vi "Measurement UI.vi"() -> ()   [LabVIEW 2025, in "Automotive Vision UI.lvlib"]
uses:
  Automotive Vision UI.lvlib
  <vilib>/gRPC/LabVIEW gRPC Library/Shared/grpcId.ctl
  <vilib>/vision/Image Controls.llb/IMAQ Image.ctl
  Automotive-Vision-OOBService_client/RPC Messages/hwval_BoolRequest.ctl
  Automotive-Vision-OOBService_client/RPC Messages/hwval_ExportRequest.ctl
  Automotive-Vision-OOBService_client/RPC Messages/hwval_ExportTypeRequest.ctl
  Automotive-Vision-OOBService_client/RPC Messages/hwval_ExportFileType.ctl
  <vilib>/gRPC/LabVIEW gRPC Library/grpc-lvsupport-release.lvlib
  Automotive-Vision-OOBService_client/Automotive-Vision-OOBService_client.lvlib
panel:
  in  "HELP":bool
  out "WIDTH":u64
  out "HEIGHT":u64
  out "Numeric":i32
  out "error out":errorcluster
  in  "GRPC status":string
  out "OOB gRPC Port":i32
  in  "BITFILE":string="IMAGE RESOLUTION: 800x600 - RAW12"
  in  "SERIAL (SI) CHANNEL":u32(ring) items=["SI0", "SI1", "SI2", "SI3"]
  out "Available SI Devices":string[][](array[string])
  in  "RIO HANDLER":string
  in  "AUTO. VISION DEVICE":u32(ring) items=["PXI1Slot2", "PXI1Slot5"]
  out "BYTES ACQUIRED":u64 format="%#.2p"
  out "ERROR":bool
  out "IMAGE PIXEL DATA":u32[](array[numeric])
  in  "IMAGE SAVE FORMAT":u32(ring) items=["PNG", "RAW LLP"]
  out "FRAME COUNT":u64
  out "IMAGE DATA":string
  in  "PAUSE":bool
  in  "CAPTURE":bool
  in  "PATH TO IMAGE CAPTURE":path=path "C:/Users/Public/Documents"
  in  "INTERPRETATION":u32(ring) items=["Grayscale", "Bayer", "RGB", "YUV422", "YUV420", "Legacy YUV420"]
  in  "PATTERN":u32(ring) items=["GB", "GR", "BG", "RG"]
  in  "ALGORITHM":u32(ring) items=["BILINEAR", "VNG"]
  in  "VIRTUAL CHANNEL":u32
  in  "PAYLOAD DATA TYPE":T1(ring)=enum."RAW 8"
  in  "SERIAL CHANNEL":string="SI1"
  out "SOURCE RATE (fps)":dbl format="%#.2f FPS"
  in  "SI ACTIVE LANE CNT":u32(ring)=4 items=["1 LANE"=1, "2 LANE"=2, "4 LANE"=4]
  in  "REF. CLOCK  (Hz)":dbl=25000000.0 format="%#_6p"
  in  "POC SOURCE":u32(ring) items=["NONE", "INTERNAL", "AUXILIARY"]
  out "STATE MESSAGE":string
  in  "CSI-2 DATA SOURCE":u32(ring) items=["CORRECTED", "RAW"]
  in  "PATH TO CONFIGURATION SCRIPT":path
  out "POC CURRENT (mA)":dbl format="%#.2pA"
  out "POC VOLTAGE (V)":dbl format="%#.0pV"
  out "ACQ. DURATION (s)":dbl format="%#.2ps"
  out "ACQ. IN PROGRESS":bool
  out "DISPLAY":T2(plugin-control)
  # "CONFIGURATION"
  # "Image path parameters"
  # "Board parameters"
  # "Display parameters"
  # "STATUS"
  # "CONTROL"
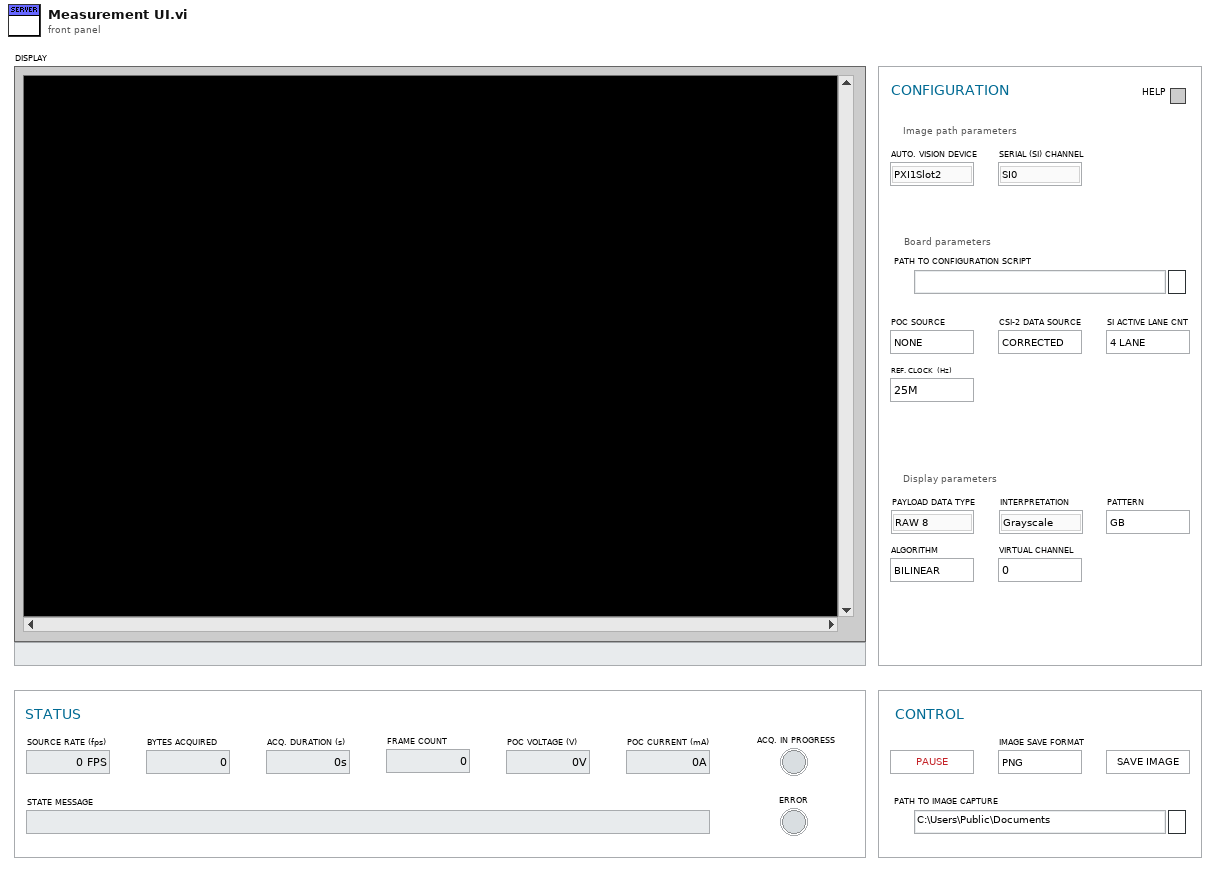
[diagram p1: front panel]
types:
  T1 = enum32{"Frame Start", "Frame End", "Line Start", "Line End", "End of Transmission", "Reserved 0", "Reserved 1", "Reserved 2", "Generic Short Packet 1", "Generic Short Packet 2", "Generic Short Packet 3", "Generic Short Packet 4", "Generic Short Packet 5", "Generic Short Packet 6", "Generic Short Packet 7", "Generic Short Packet 8", "Null", "Blanking Data", "Embedded 8-bit non Image Data", "Generic Long Packet 1", "Generic Long Packet 2", "Generic Long Packet 3", "Generic Long Packet 4", "Reserved 3", "YUV420 8-bit", "YUV420 10-bit", "Legacy YUV420 8-bit", "Reserved 4", "YUV420 8-bit Chroma Shifted", "YUV420 10-bit Chroma Shifted", "YUV422 8-bit", "YUV422 10-bit", "RGB444", "RGB555", "RGB565", "RGB666", "RGB888", "Reserved 5", "Reserved 6", "RAW 24", "RAW 6", "RAW 7", "RAW 8", "RAW 10", "RAW 12", "RAW 14", "RAW 16", "RAW 20", "User Defined 8-bit Data 1", "User Defined 8-bit Data 2", "User Defined 8-bit Data 3", "User Defined 8-bit Data 4", "User Defined 8-bit Data 5", "User Defined 8-bit Data 6", "User Defined 8-bit Data 7", "User Defined 8-bit Data 8", "USL Command", "Reserved 7", "Reserved 8", "Reserved 9", "Reserved 10", "Reserved 11", "Reserved 12", "LRTE EPD Spacer"}
  T2 = typedef "IMAQ Image.ctl" = refnum<image>
  T3 = typedef "grpc-lvsupport-release.lvlib/grpcId.ctl" = u64
  T4 = typedef "Automotive-Vision-OOBService_client.lvlib/hwval_BoolRequest.ctl" = cluster{"BooleanData":bool}
  T5 = typedef "Automotive-Vision-OOBService_client.lvlib/hwval_ExportRequest.ctl" = cluster{"FilePath":string}
  T6 = typedef "Automotive-Vision-OOBService_client.lvlib/hwval_ExportTypeRequest.ctl" = cluster{"FileType":T7}
  T7 = typedef "Automotive-Vision-OOBService_client.lvlib/hwval_ExportFileType.ctl" = enum32{"EXPORT_PNG", "EXPORT_RAW"}
  T8 = enum8{"Enabled", "Disabled", "Disabled and Grayed Out"}
  T9 = cluster{"pattern":i32, "algorithm":i32, "red gain":dbl, "green gain":dbl, "blue gain":dbl}
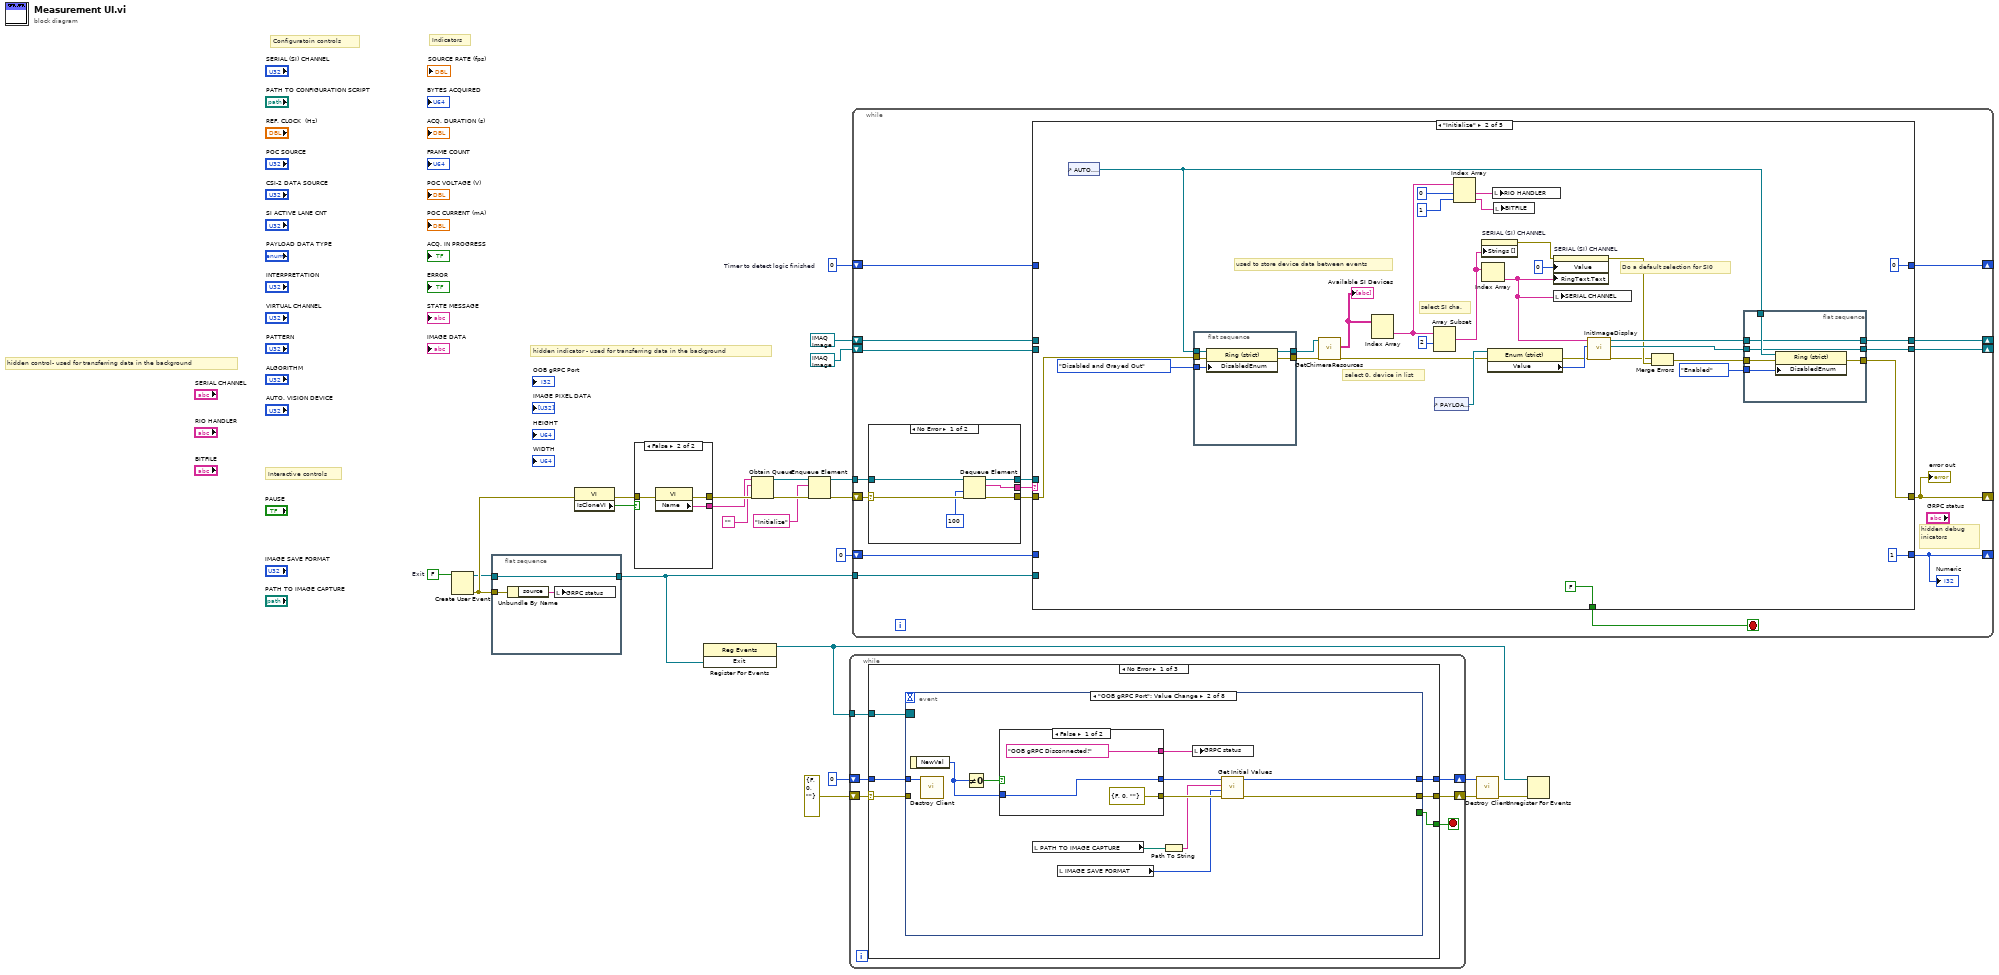
[diagram p0: block diagram]
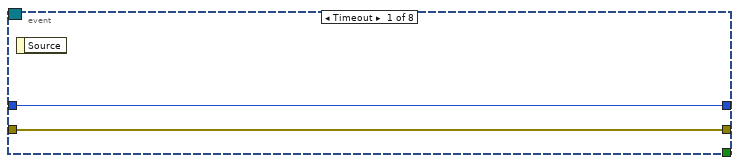
[diagram p2: hidden frame]
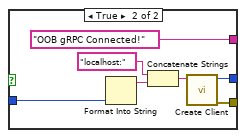
[diagram p3: hidden frame]
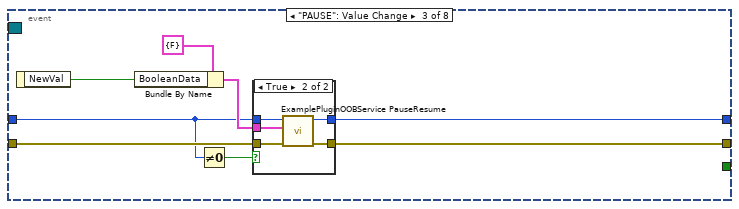
[diagram p4: hidden frame]
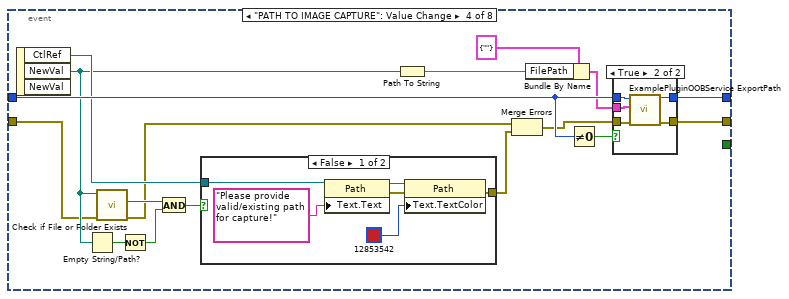
[diagram p6: hidden frame]
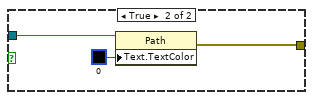
[diagram p7: hidden frame]
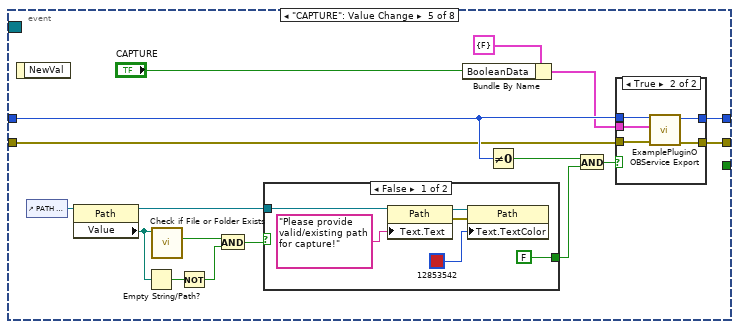
[diagram p9: hidden frame]
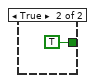
[diagram p10: hidden frame]
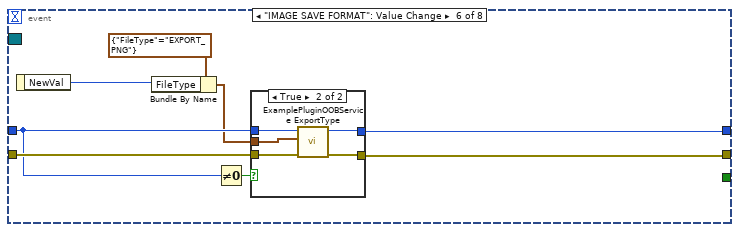
[diagram p12: hidden frame]
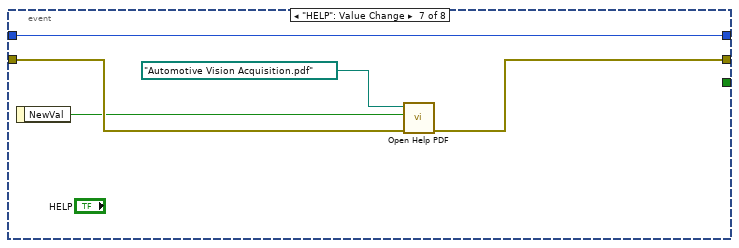
[diagram p14: hidden frame]
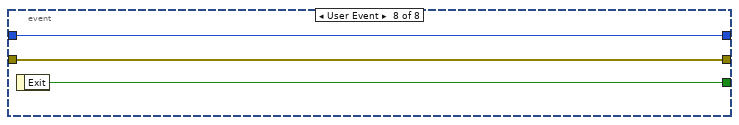
[diagram p15: hidden frame]
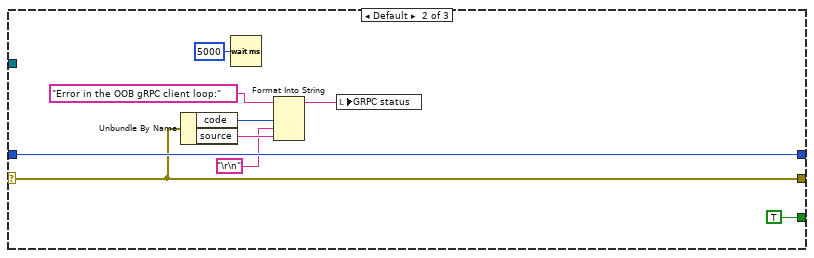
[diagram p16: hidden frame]
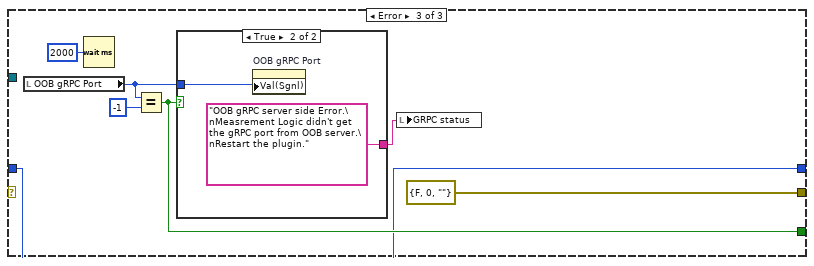
[diagram p17: hidden frame]
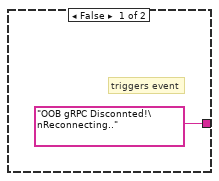
[diagram p18: hidden frame]
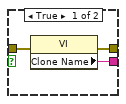
[diagram p19: hidden frame]
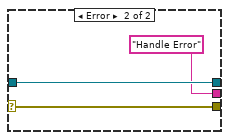
[diagram p20: hidden frame]
diagram:
  w5 = 0  # Timer to detect logic finished
  w14 = FALSE  # Exit
  # "Indicators"
  # "Configuratoin controls"
  # "Interactive controls"
  # "hidden indicator - used for transferring data in the background"
  # "hidden control- used for transferring data in the background"
  n1 = Create User Event(user event datatype=w14) -> (user event=w1:refnum<user-event>, error out=w7:errorcluster)  [unwired: 1 in]
  n2 = flat-sequence {
    tunnel: [w27] -> w8
    tunnel: w1 -> [w27]
    tunnel: w7 -> [w26]
    frame #0 {
      n3 = Unbundle By Name(w26) -> ("source"=w25:string)
      n4 = local write "GRPC status"(w25) -> ()
    }
  }
  n5 = property on="Property Node" class="VI"(error in=w7) -> (error out=w15:errorcluster, "IsCloneVI"=w16:bool)  [unwired: 1 in, 1 out]
  n6 = case shown="False" w16 {
    tunnel: [w30 w33] -> w24
    tunnel: [w29 w32] -> w23
    tunnel: w15 -> [w28 w31]
    frame True {
      n7 = property on="Property Node" class="VI"(error in=w28) -> (error out=w30:errorcluster, "Clone Name"=w29:string)  [unwired: 1 in, 1 out]
    }
    frame False {
      n8 = property on="Property Node" class="VI"(error in=w31) -> (error out=w33:errorcluster, "Name"=w32:string)  [unwired: 1 in, 1 out]
    }
  }
  n9 = register-events(w8) -> (reference out=w13:refnum<event-registration>)  [unwired: 2 in, 1 out]
  n10 = Obtain Queue(name (unnamed)=w23, element data type="" ("Empty String Constant"), error in (no error)=w24) -> (queue out=w20:refnum<queue>, error out=w22:errorcluster)  [unwired: 2 in, 1 out]
  n11 = Enqueue Element(queue=w20, element="Initialize", error in (no error)=w22) -> (queue out=w19:refnum<queue>, error out=w21:errorcluster)  [unwired: 1 in, 1 out]
  n12 = while {
    tunnel: w13 -> [w36]
    shift-right: [w37] -> w11
    shift-left: errorcluster {"status"=FALSE, "code"=0, "source"=""} ("error IO") -> [w39]
    shift-right: [w34] -> w9
    shift-left: T3 0 ("gRPC ID out") -> [w35]
    stop <- w38 stop-if-true
    n13 = case shown="No Error" w39 {
      selector: w39 -> [w43 w172 _]
      tunnel: [w40 TRUE w184] -> w38
      tunnel: [w44 w172 errorcluster {"status"=FALSE, "code"=0, "source"=""} ("error IO")] -> w37
      tunnel: w36 -> [w45 _ _]
      tunnel: w35 -> [w42 w177 w182]
      tunnel: [w41 w177 w182] -> w34
      frame No Error {
        n14 = event shown="[1] \"OOB gRPC Port\": Value Change" {
          selector: w45 -> [_ _ _ _ _ _ _ _]
          dyn-events: _ -> [_ _ _ _ _ _ _ _]
          timeout: _ -> [_ _ _ _ _ _ _ _]
          tunnel: [w47 w52 w74 w98 w132 w152 w164 w167] -> w44
          tunnel: w43 -> [w47 _ w73 w83 w126 w153 w165 w167]
          tunnel: w42 -> [w46 w54 w69 w96 w131 w151 w166 w168]
          tunnel: [w46 w51 w75 w99 w130 w150 w166 w168] -> w41
          tunnel: [_ _ _ _ _ _ _ w169] -> w40
          event Timeout {
            n15 = event-data() -> ()  [unwired: 1 in, 1 out]
          }
          event "OOB gRPC Port": Value Change {
            n16 = event-data() -> ("NewVal"=w55:i32)  [unwired: 1 in]
            n17 = call "Destroy Client.vi"("gRPC ID"=w54) -> ()  [unwired: 10 in, 1 out]
            n18 = Not Equal To 0?(x=w55) -> (x != 0?=w56:bool)
            n19 = case shown="False" w56 {
              tunnel: [errorcluster {"status"=FALSE, "code"=0, "source"=""} ("error out") w61] -> w57
              tunnel: w55 -> [w60 w65]
              tunnel: [w60 w62] -> w51
              tunnel: ["OOB gRPC Disconnected!" ("Status") "OOB gRPC Connected!" ("Status")] -> w53
              frame False {
              }
              frame True {
                n20 = Format Into String(w65) -> (resulting string=w67:string)  [unwired: 3 in, 1 out]
                n21 = Concatenate Strings("localhost:" ("string"), w67) -> (w63:string)
                n22 = call "Create Client.vi"("address"=w63) -> ("error out"=w61:errorcluster, "gRPC ID Out"=w62:T3)  [unwired: 9 in]
              }
            }
            n23 = local read "PATH TO IMAGE CAPTURE"() -> (w49:path)
            n24 = local read "IMAGE SAVE FORMAT"() -> (w50:u32)
            n25 = Path To String(path=w49) -> (string=w48:string)
            n26 = local write "GRPC status"(w53) -> ()
            n27 = call "Get Initial Values.vi"("error in"=w57, "IMAGE SAVE FORMAT"=w50, "String"=w48, "gRPC ID In"=w51) -> ("error out"=w52:errorcluster)  [unwired: 7 in]
          }
          event "PAUSE": Value Change {
            n28 = event-data() -> ("NewVal"=w71:bool)  [unwired: 1 in]
            n29 = Bundle By Name(cluster=T4 {"BooleanData"=FALSE} ("Request Data"), "BooleanData"=w71) -> (w72:T4)
            n30 = Not Equal To 0?(x=w69) -> (x != 0?=w70:bool)
            n31 = case shown="True" w70 {
              tunnel: [w77 w81] -> w75
              tunnel: [w76 w80] -> w74
              tunnel: w69 -> [w77 w82]
              tunnel: w73 -> [w76 w79]
              tunnel: w72 -> [_ w78]
              frame False {
              }
              frame True {
                n32 = call "ExamplePluginOOBService PauseResume.vi"("error in"=w79, "Request Data"=w78, "gRPC ID"=w82) -> ("error out"=w80:errorcluster, "gRPC ID out"=w81:T3)  [unwired: 6 in, 1 out]
              }
            }
          }
          event "PATH TO IMAGE CAPTURE": Value Change {
            n33 = event-data() -> ("CtlRef"=w92:refnum<vi>, "NewVal"=w88:path)  [unwired: 1 in, 1 out]
            n34 = Empty String/Path?(string/path=w88) -> (empty?=w91:bool)
            n35 = call <vilib>:"Check if File or Folder Exists.vi"("error in (no error)"=w83, "path"=w88) -> ("error out"=w84:errorcluster, "file or folder exists?"=w90:bool)  [unwired: 7 in, 1 out]
            n36 = Not(x=w91) -> (.not. x?=w89:bool)
            n37 = And(x=w90, y=w89) -> (x .and. y?=w87:bool)
            n38 = case shown="False" w87 {
              tunnel: w92 -> [w105 w108]
              tunnel: [w100 w106] -> w85
              frame False {
                n39 = property on="Property Node" class="Path"(reference=w105, "Text.Text"="Please provide valid/existing path for capture!" ("Path Text.Text")) -> (reference out=w104:refnum<vi>, error out=w103:errorcluster)  [unwired: 1 in]
                n40 = property on="Property Node" class="Path"(reference=w104, error in=w103, "Text.TextColor"=u32 12853542 ("Path Text.Text Colors:Text Color")) -> (error out=w100:errorcluster)  [unwired: 1 out]
              }
              frame True {
                n41 = property on="Property Node" class="Path"(reference=w108, "Text.TextColor"=u32 0 ("Path Text.Text Colors:Text Color")) -> (error out=w106:errorcluster)  [unwired: 1 in, 1 out]
              }
            }
            n42 = Path To String(path=w88) -> (string=w94:string)
            n43 = Merge Errors(w84, w85) -> (w86:errorcluster)
            n44 = Bundle By Name(cluster=T5 {"FilePath"=""} ("Request Data"), "FilePath"=w94) -> (w93:T5)
            n45 = Not Equal To 0?(x=w96) -> (x != 0?=w97:bool)
            n46 = case shown="True" w97 {
              tunnel: [w110 w114] -> w99
              tunnel: [w109 w112] -> w98
              tunnel: w96 -> [w110 w115]
              tunnel: w86 -> [w109 w113]
              tunnel: w93 -> [_ w111]
              frame False {
              }
              frame True {
                n47 = call "ExamplePluginOOBService ExportPath.vi"("error in"=w113, "Request Data"=w111, "gRPC ID"=w115) -> ("error out"=w112:errorcluster, "gRPC ID out"=w114:T3)  [unwired: 6 in, 1 out]
              }
            }
          }
          event "CAPTURE": Value Change {
            n48 = event-data() -> ()  [unwired: 1 in, 1 out]
            n49 = control-ref of="PATH TO IMAGE CAPTURE"() -> (w122:refnum<vi>)
            n50 = property on="Property Node" class="Path"(reference=w122) -> (reference out=w127:refnum<vi>, "Value"=w121:path)  [unwired: 1 in, 1 out]
            n51 = Empty String/Path?(string/path=w121) -> (empty?=w120:bool)
            n52 = call <vilib>:"Check if File or Folder Exists.vi"("path"=w121) -> ("file or folder exists?"=w118:bool)  [unwired: 8 in, 2 out]
            n53 = Not(x=w120) -> (.not. x?=w117:bool)
            n54 = And(x=w118, y=w117) -> (x .and. y?=w119:bool)
            n55 = case shown="False" w119 {
              tunnel: w127 -> [w138 _]
              tunnel: [FALSE TRUE] -> w123
              frame False {
                n56 = property on="Property Node" class="Path"(reference=w138, "Text.Text"="Please provide valid/existing path for capture!" ("Path Text.Text")) -> (reference out=w137:refnum<vi>, error out=w136:errorcluster)  [unwired: 1 in]
                n57 = property on="Property Node" class="Path"(reference=w137, error in=w136, "Text.TextColor"=u32 12853542 ("Path Text.Text Colors:Text Color")) -> ()  [unwired: 2 out]
              }
              frame True {
              }
            }
            n58 = Bundle By Name(cluster=T4 {"BooleanData"=FALSE} ("Request Data"), "BooleanData"="CAPTURE") -> (w128:T4)
            n59 = Not Equal To 0?(x=w131) -> (x != 0?=w125:bool)
            n60 = And(x=w125, y=w123) -> (x .and. y?=w124:bool)
            n61 = case shown="True" w124 {
              tunnel: w126 -> [w140 w146]
              tunnel: [w140 w145] -> w132
              tunnel: w131 -> [w141 w144]
              tunnel: [w141 w143] -> w130
              tunnel: w128 -> [_ w142]
              frame False {
              }
              frame True {
                n62 = call "ExamplePluginOOBService Export.vi"("error in"=w146, "Request Data"=w142, "gRPC ID"=w144) -> ("error out"=w145:errorcluster, "gRPC ID out"=w143:T3)  [unwired: 6 in, 1 out]
              }
            }
          }
          event "IMAGE SAVE FORMAT": Value Change {
            n63 = event-data() -> ("NewVal"=w148:u32)  [unwired: 1 in]
            n64 = Bundle By Name(cluster=T6 {"FileType"=enum."EXPORT_PNG"} ("Request Data"), "FileType"=w148) -> (w147:T6)
            n65 = Not Equal To 0?(x=w151) -> (x != 0?=w154:bool)
            n66 = case shown="True" w154 {
              tunnel: w153 -> [w155 w159]
              tunnel: [w155 w158] -> w152
              tunnel: w151 -> [w156 w160]
              tunnel: [w156 w157] -> w150
              tunnel: w147 -> [_ w161]
              frame False {
              }
              frame True {
                n67 = call "ExamplePluginOOBService ExportType.vi"("error in"=w159, "Request Data"=w161, "gRPC ID"=w160) -> ("error out"=w158:errorcluster, "gRPC ID out"=w157:T3)  [unwired: 6 in, 1 out]
              }
            }
          }
          event "HELP": Value Change {
            n68 = event-data() -> ("NewVal"=w163:bool)  [unwired: 1 in]
            n69 = call "Open Help PDF.vi"("error in"=w165, "NewVal"=w163, "Path after documentation"=path "Automotive Vision Acquisition.pdf") -> ("error out"=w164:errorcluster)  [unwired: 8 in]
          }
          event User Event {
            n70 = event-data() -> ("Exit"=w169:bool)  [unwired: 1 in]
          }
        }
      }
      frame Default {
        n71 = Unbundle By Name(w172) -> ("code"=w176:i32, "source"=w175:string)
        n72 = Wait (ms)(milliseconds to wait=u32 5000) -> ()  [unwired: 1 out]
        n73 = Format Into String(initial string="Error in the OOB gRPC client loop:" ("format string"), w176, "\r\n" ("End of Line Constant"), w175) -> (resulting string=w170:string)  [unwired: 2 in, 1 out]
        n74 = local write "GRPC status"(w170) -> ()
      }
      frame Error {
        n75 = local read "OOB gRPC Port"() -> (w180:i32)
        n76 = Wait (ms)(milliseconds to wait=u32 2000) -> ()  [unwired: 1 out]
        n77 = Equal?(x=w180, y=-1 ("x")) -> (x = y?=w184:bool)
        n78 = case shown="True" w184 {
          tunnel: ["OOB gRPC Disconnted!\nReconnecting.." ("Status") "OOB gRPC server side Error.\nMeasrement Logic didn't get the gRPC port from OOB server.\nRestart the plugin." ("Status")] -> w179
          tunnel: w180 -> [_ w187]
          frame False {
            # "triggers event"
          }
          frame True {
            n79 = property on="OOB gRPC Port" class="DigNum (strict)"("Val(Sgnl)"=w187) -> ()  [unwired: 2 in, 2 out]
          }
        }
        n80 = local write "GRPC status"(w179) -> ()
      }
    }
  }
  n81 = while {
    shift-right: [w193] -> _
    shift-left: w21 -> [w204]
    tunnel: w19 -> [w202]
    shift-right: [w195] -> _
    shift-left: T2 refnum ("Image Out Grayscale") -> [w197]
    shift-right: [w198] -> _
    shift-left: T2 refnum ("Image Out Grayscale") -> [w196]
    tunnel: w8 -> [w194]
    shift-right: [w191] -> _
    shift-left: 0 -> [w192]
    shift-right: [w189] -> _
    shift-left: w5 -> [w190]
    stop <- w199 stop-if-true
    # "hidden debug inicators"
    n82 = case shown="No Error" w204 {
      selector: w204 -> [w210 w213]
      tunnel: [w209 w213] -> w203
      tunnel: w202 -> [w208 w212]
      tunnel: [w207 w212] -> w201
      tunnel: [w206 "Handle Error"] -> w200
      frame No Error {
        n83 = Dequeue Element(queue=w208, timeout in ms (-1)=100, error in (no error)=w210) -> (queue out=w207:refnum<queue>, element=w206:string, error out=w209:errorcluster)  [unwired: 1 out]
      }
      frame Error {
      }
    }
    n84 = case shown="\"Initialize\"" w200 {
      tunnel: w203 -> [w226 w342 w363 w413 w451]
      tunnel: w201 -> [w224 _ _ w436 w450]
      tunnel: [w227 w341 w399 w407 w449] -> w193
      tunnel: [_ FALSE _ TRUE TRUE] -> w199
      tunnel: [w222 w335 w402 w429 w456] -> w198
      tunnel: [w223 w333 w400 w429 w457] -> w195
      tunnel: w197 -> [w221 _ w400 w430 w457]
      tunnel: w196 -> [w220 _ w402 w431 w456]
      tunnel: w194 -> [_ _ _ w417 _]
      tunnel: w192 -> [_ _ w380 _ _]
      tunnel: [-3 1 w379 -1 -2] -> w191
      tunnel: [w214 0 ("Numeric 2") 0 ("Numeric 2") 0 ("Numeric 2") 0 ("Numeric 2")] -> w189
      tunnel: w190 -> [w215 _ _ _ _]
      frame "Event", Default {
        n85 = event shown="[0] Timeout" {
          selector: _ -> [_ _ _ _ _]
          dyn-events: _ -> [_ _ _ _ _]
          timeout: 100 -> [_ _ _ _ _]
          tunnel: [w228 w263 w297 w308 w315] -> w227
          tunnel: w226 -> [w231 _ w304 w308 w316]
          tunnel: w224 -> [w230 _ _ _ w314]
          tunnel: w221 -> [_ w266 w302 w307 w312]
          tunnel: w220 -> [_ w267 w303 w306 w311]
          tunnel: [_ w266 w299 w307 w312] -> w219
          tunnel: [_ w267 w298 w306 w311] -> w217
          tunnel: [_ _ TRUE _ _] -> w218
          tunnel: w215 -> [w237 _ _ _ _]
          tunnel: [w236 _ _ _ _] -> w214
          event Timeout {
            n86 = event-data() -> ()  [unwired: 1 in, 3 out]
            n87 = control-ref of="ACQ. IN PROGRESS"() -> (w233:refnum<vi>)
            n88 = Increment(x=w237) -> (x+1=w236:i32)
            n89 = property on="Property Node" class="Bool (strict)"(reference=w233) -> ("Value"=w232:bool)  [unwired: 1 in, 2 out]
            n90 = Greater?(x=w236, y=10) -> (0:w234:bool)
            n91 = And(x=w234, y=w232) -> (x .and. y?=w229:bool)
            n92 = case shown="True" w229 {
              tunnel: w231 -> [w238 w240]
              tunnel: w230 -> [_ _]
              tunnel: [w238 w242] -> w228
              frame False {
              }
              frame True {
                # "Only update status to done if no error happend"
                n93 = control-ref of="ACQ. IN PROGRESS"() -> (w243:refnum<vi>)
                n94 = property on="Property Node" class="Bool (strict)"(reference=w243, error in=w240, "Value"=FALSE) -> (error out=w239:errorcluster)  [unwired: 1 out]
                n95 = control-ref of="STATE MESSAGE"() -> (w244:refnum<vi>)
                n96 = property on="Property Node" class="Str"(reference=w244, error in=w239) -> (reference out=w252:refnum<vi>, error out=w246:errorcluster, "Value"=w251:string)
                n97 = Search and Replace String(case sensitive?=TRUE ("ignore case? (F)"), input string=w251, search string="error", error in=w246) -> (number of replacements=w248:i32, error out=w245:errorcluster)  [unwired: 4 in, 2 out]
                n98 = Equal To 0?(x=w248) -> (x = 0?=w247:bool)
                n99 = case shown="True" w247 {
                  tunnel: w252 -> [_ w259]
                  tunnel: w251 -> [_ w257]
                  tunnel: w245 -> [w253 w255]
                  tunnel: [w253 w256] -> w242
                  frame False {
                  }
                  frame True {
                    n100 = Search and Replace String(input string=w257, search string="^.*", replace string="Done" ("replace string (\"\")"), error in=w255) -> (result string=w258:string, error out=w254:errorcluster)  [unwired: 4 in, 2 out]
                    n101 = property on="Property Node" class="Str"(reference=w259, error in=w254, "Value"=w258) -> (error out=w256:errorcluster)  [unwired: 1 out]
                  }
                }
              }
            }
          }
          event "AUTO. VISION DEVICE": Value Change {
            n102 = event-data() -> ("CtlRef"=w274:refnum<vi>)  [unwired: 1 in, 5 out]
            n103 = property on="Property Node" class="Ring (strict)"(reference=w274) -> (error out=w265:errorcluster, "RingText.Text"=w272:string)  [unwired: 1 in, 1 out]
            n104 = local read "Available SI Devices"() -> (w273:string[][])
            n105 = for {
              tunnel: w273 -> [w284] mode=indexing
              tunnel: w272 -> [w287]
              tunnel: [w286] -> w270
              tunnel: [w282] -> w262
              stop <- w285 stop-if-true
              n106 = Index Array(array=w284) -> (element=w288:string)  [unwired: 1 in]
              n107 = Index Array(array=w284, index=1) -> (element=w282:string)
              n108 = Equal?(x=w287, y=w288) -> (x = y?=w285:bool)
              n109 = case shown="True" w285 {
                tunnel: w284 -> [_ w292]
                tunnel: [string[] [] w290] -> w286
                frame False {
                }
                frame True {
                  n110 = Array Subset(array=w292, index=2) -> (w290:string[])  [unwired: 1 in]
                }
              }
            }
            n111 = local write "RIO HANDLER"(w272) -> ()
            n112 = property on="SERIAL (SI) CHANNEL" class="Ring (strict)"(error in=w265) -> (error out=w264:errorcluster, "Strings []"=w271:string[])  [unwired: 1 in, 1 out]
            n113 = local write "BITFILE"(w262) -> ()
            n114 = Not Equal?(x=w271, y=w270) -> (x != y?=w269:bool[])
            n115 = And Array Elements(Boolean array=w269) -> (logical AND=w268:bool)
            n116 = case shown="True" w268 {
              tunnel: w270 -> [_ w278]
              tunnel: w264 -> [w275 w277]
              tunnel: [w275 w276] -> w263
              frame False {
              }
              frame True {
                n117 = Index Array(array=w278) -> (element=w280:string)  [unwired: 1 in]
                n118 = property on="SERIAL (SI) CHANNEL" class="Ring (strict)"(error in=w277, "Strings []"=w278) -> (error out=w281:errorcluster)  [unwired: 1 in, 1 out]
                n119 = local write "SERIAL CHANNEL"(w280) -> ()
                n120 = property on="SERIAL (SI) CHANNEL" class="Ring (strict)"(error in=w281, "Value"=0, "RingText.Text"=w280) -> (error out=w276:errorcluster)  [unwired: 1 in, 1 out]
              }
            }
          }
          event "PAYLOAD DATA TYPE": Value Change {
            n121 = event-data() -> ("CtlRef"=w301:refnum<vi>)  [unwired: 1 in, 5 out]
            n122 = call "IMAQ Dispose"("Image"=w303, "error in (no error)"=w304) -> ("error out"=w305:errorcluster)  [unwired: 4 in]
            n123 = call "IMAQ Dispose"("Image"=w302, "error in (no error)"=w305) -> ("error out"=w294:errorcluster)  [unwired: 4 in]
            n124 = property on="Property Node" class="Enum (strict)"(reference=w301, error in=w294) -> (error out=w293:errorcluster, "Value"=w295:T1)  [unwired: 1 out]
            n125 = local read "SERIAL CHANNEL"() -> (w300:string)
            n126 = call "InitImageDisplay.vi"("error in (no error)"=w293, "payload data type"=w295, "SI channel"=w300) -> ("error out"=w297:errorcluster, "Image Out Color"=w298:T2, "Image Out Grayscale"=w299:T2)  [unwired: 6 in]
          }
          event "SERIAL (SI) CHANNEL": Value Change {
            n127 = event-data() -> ("CtlRef"=w310:refnum<vi>)  [unwired: 1 in, 5 out]
            n128 = property on="Property Node" class="Ring (strict)"(reference=w310) -> ("RingText.Text"=w309:string)  [unwired: 1 in, 2 out]
            n129 = local write "SERIAL CHANNEL"(w309) -> ()
          }
          event Panel Close? {
            n130 = event-data() -> ()  [unwired: 1 in, 4 out]
            n131 = Enqueue Element(queue=w314, element="Exit", error in (no error)=w316) -> (error out=w315:errorcluster)  [unwired: 1 in, 2 out]
            n132 = event-data ("Event Filter Node")("Discard?"=TRUE) -> ()  [unwired: 1 in, 1 out]
          }
        }
        n133 = Select(t=w219, s=w218, f=w221) -> (s? t:f=w223:T2)
        n134 = Select(t=w217, s=w218, f=w220) -> (s? t:f=w222:T2)
      }
      frame "Initialize" {
        # "Do a default selection for SI0"
        # "select SI cha."
        # "select 0. device in list"
        # "used to store device data between events"
        n135 = control-ref of="AUTO. VISION DEVICE"() -> (w340:refnum<vi>)
        n136 = flat-sequence {
          tunnel: [w358] -> w343
          tunnel: w340 -> [w360]
          tunnel: [w356] -> w324
          tunnel: w342 -> [w357]
          tunnel: T8."Disabled and Grayed Out" ("Disabled") -> [w359]
          frame #0 {
            n137 = property on="Property Node" class="Ring (strict)"(reference=w360, error in=w357, "DisabledEnum"=w359) -> (reference out=w358:refnum<vi>, error out=w356:errorcluster)
          }
        }
        n138 = call "GetChimeraResources.vi"("error in (no error)"=w324, "Automotive Vision Device selector"=w343) -> ("error out"=w323:errorcluster, "Available input channels on Automotive Camera Vision Devices"=w346:string[][])  [unwired: 6 in, 2 out]
        "Available SI Devices" <- w346
        n139 = Index Array(array=w346) -> (element=w337:string[])  [unwired: 2 in]
        n140 = Array Subset(array=w337, index=2) -> (w345:string[])  [unwired: 1 in]
        n141 = control-ref of="PAYLOAD DATA TYPE"() -> (w331:refnum<vi>)
        n142 = Index Array(array=w337, index #1=0 ("index"), index #2=1 ("index")) -> (element #1=w338:string, element #2=w325:string)
        n143 = property on="SERIAL (SI) CHANNEL" class="Ring (strict)"("Strings []"=w345) -> (error out=w348:errorcluster)  [unwired: 2 in, 1 out]
        n144 = Index Array(array=w345) -> (element=w336:string)  [unwired: 1 in]
        n145 = property on="Property Node" class="Enum (strict)"(reference=w331, error in=w323) -> (error out=w322:errorcluster, "Value"=w330:T1)  [unwired: 1 out]
        n146 = local write "RIO HANDLER"(w338) -> ()
        n147 = local write "BITFILE"(w325) -> ()
        n148 = property on="SERIAL (SI) CHANNEL" class="Ring (strict)"(error in=w348, "Value"=0, "RingText.Text"=w336) -> (error out=w321:errorcluster)  [unwired: 1 in, 1 out]
        n149 = local write "SERIAL CHANNEL"(w336) -> ()
        n150 = call "InitImageDisplay.vi"("error in (no error)"=w322, "payload data type"=w330, "SI channel"=w336) -> ("error out"=w320:errorcluster, "Image Out Color"=w334:T2, "Image Out Grayscale"=w332:T2)  [unwired: 6 in]
        n151 = Merge Errors(w320, w321) -> (w319:errorcluster)
        n152 = flat-sequence {
          tunnel: [w351] -> w341
          tunnel: w319 -> [w352]
          tunnel: w340 -> [w355]
          tunnel: [w354] -> w335
          tunnel: w334 -> [w354]
          tunnel: [w353] -> w333
          tunnel: w332 -> [w353]
          tunnel: T8."Enabled" ("Disabled") -> [w350]
          frame #0 {
            n153 = property on="Property Node" class="Ring (strict)"(reference=w355, error in=w352, "DisabledEnum"=w350) -> (error out=w351:errorcluster)  [unwired: 1 out]
          }
        }
      }
      frame "Post UI Update" {
        w396 = 1.0 ("red gain")
        # "Generate an event when grpc port value is not equal to 0 and it has changed."
        # "This case will be triggered, after framework updates the User interface with result values."
        n154 = control-ref of="WIDTH"() -> (w376:refnum<vi>)
        n155 = control-ref of="HEIGHT"() -> (w375:refnum<vi>)
        n156 = control-ref of="PAYLOAD DATA TYPE"() -> (w394:refnum<vi>)
        n157 = control-ref of="IMAGE PIXEL DATA"() -> (w403:refnum<vi>)
        n158 = control-ref of="INTERPRETATION"() -> (w393:refnum<vi>)
        n159 = control-ref of="PATTERN"() -> (w392:refnum<vi>)
        n160 = control-ref of="ALGORITHM"() -> (w390:refnum<vi>)
        n161 = property on="Property Node" class="Enum (strict)"(reference=w394) -> (error out=w370:errorcluster, "Value"=w378:T1)  [unwired: 1 in, 1 out]
        n162 = property on="Property Node" class="Arr (strict)"(reference=w403) -> (error out=w369:errorcluster, "Value"=w398:u32[])  [unwired: 1 in, 1 out]
        n163 = property on="Property Node" class="DigNum (strict)"(reference=w376) -> (error out=w368:errorcluster, "Value"=w374:u64)  [unwired: 1 in, 1 out]
        n164 = property on="Property Node" class="DigNum (strict)"(reference=w375) -> (error out=w367:errorcluster, "Value"=w372:u64)  [unwired: 1 in, 1 out]
        n165 = property on="Property Node" class="Ring (strict)"(reference=w393) -> (error out=w366:errorcluster, "Value"=w377:u32)  [unwired: 1 in, 1 out]
        n166 = property on="Property Node" class="Ring (strict)"(reference=w392) -> (error out=w365:errorcluster, "Value"=w391:u32)  [unwired: 1 in, 1 out]
        n167 = property on="Property Node" class="Ring (strict)"(reference=w390) -> (error out=w364:errorcluster, "Value"=w389:u32)  [unwired: 1 in, 1 out]
        n168 = Merge Errors(w363, w370, w369, w368, w367, w366, w365, w364) -> (w362:errorcluster)
        n169 = Bundle By Name(cluster=T9 {"pattern"=0, "algorithm"=0, "red gain"=0.0, "green gain"=0.0, "blue gain"=0.0} ("bayer parameters"), "pattern"=w391, "algorithm"=w389, "red gain"=w396, "green gain"=w396, "blue gain"=w396) -> (w395:T9)
        n170 = To Unsigned Word Integer(number=w374) -> (unsigned 16bit integer=w373:u16)
        n171 = To Unsigned Word Integer(number=w372) -> (unsigned 16bit integer=w371:u16)
        n172 = call "DisplayImage.vi"("image color"=w402, "Image Pixel Data"=w398, "data type"=w378, "Image grayscale"=w400, "width"=w373, "error in (no error)"=w362, "height"=w371, "interpretation"=w377, "bayer parameters"=w395) -> ("display image"=→"DISPLAY":T2, "error out"=w399:errorcluster)  [unwired: 5 in]
        n173 = local read "OOB gRPC Port"() -> (w382:i32)
        n174 = feedback #1(0 ("OOB gRPC Port")) -> (w385:i32)
        n175 = feedback-in #1(w382) -> ()
        n176 = Not Equal?(x=w382, y=w385) -> (x != y?=w386:bool)
        n177 = Not Equal To 0?(x=w382) -> (x != 0?=w387:bool)
        n178 = Format Into String(format string="%d Data received , port: %d" ("GRPC status"), w380, w382) -> (resulting string=w381:string)  [unwired: 2 in, 1 out]
        n179 = Compound Arithmetic op=AND(w387, w386) -> (w384:bool)
        n180 = local write "GRPC status"(w381) -> ()
        n181 = Increment(x=w380) -> (x+1=w379:i32)
        n182 = case shown="True" w384 {
          tunnel: w382 -> [_ w404]
          frame False {
          }
          frame True {
            n183 = property on="OOB gRPC Port" class="DigNum (strict)"("Val(Sgnl)"=w404) -> ()  [unwired: 2 in, 2 out]
          }
        }
      }
      frame "Exit" {
        w429 = T2 refnum ("Image Out Grayscale")
        # "Only update status to done if no error happend"
        # "This case is triggered to close the User Interface from framework"
        n184 = call "IMAQ Dispose"("Image"=w431) -> ("error out"=w432:errorcluster)  [unwired: 5 in]
        n185 = Flush Queue(queue=w436, error in (no error)=w413) -> (queue out=w435:refnum<queue>, error out=w434:errorcluster)  [unwired: 1 out]
        n186 = Generate User Event(user event=w417, event data cluster=TRUE ("event data")) -> (user event out=w418:refnum<user-event>, error out=w405:errorcluster)  [unwired: 2 in]
        n187 = call "IMAQ Dispose"("Image"=w430, "error in (no error)"=w432) -> ("error out"=w412:errorcluster)  [unwired: 4 in]
        n188 = Release Queue(queue=w435, force destroy? (F)=TRUE, error in (no error)=w434) -> (error out=w416:errorcluster)  [unwired: 2 out]
        n189 = Destroy User Event(user event=w418, error in=w405) -> (error out=w415:errorcluster)
        n190 = Merge Errors(w412, w416, w415) -> (w411:errorcluster)
        n191 = control-ref of="ACQ. IN PROGRESS"() -> (w428:refnum<vi>)
        n192 = property on="Property Node" class="Bool (strict)"(reference=w428, error in=w411, "Value"=FALSE) -> (error out=w410:errorcluster)  [unwired: 1 out]
        n193 = control-ref of="STATE MESSAGE"() -> (w426:refnum<vi>)
        n194 = property on="Property Node" class="Str"(reference=w426, error in=w410) -> (reference out=w425:refnum<vi>, error out=w409:errorcluster, "Value"=w424:string)
        n195 = Search and Replace String(case sensitive?=TRUE ("ignore case? (F)"), input string=w424, search string="error", error in=w409) -> (number of replacements=w421:i32, error out=w408:errorcluster)  [unwired: 4 in, 2 out]
        n196 = Equal To 0?(x=w421) -> (x = 0?=w420:bool)
        n197 = case shown="True" w420 {
          tunnel: w425 -> [_ w444]
          tunnel: w424 -> [_ w442]
          tunnel: w408 -> [w438 w440]
          tunnel: [w438 w441] -> w407
          frame False {
          }
          frame True {
            n198 = Search and Replace String(input string=w442, search string="^.*", replace string="Done" ("replace string (\"\")"), error in=w440) -> (result string=w443:string, error out=w439:errorcluster)  [unwired: 4 in, 2 out]
            n199 = property on="Property Node" class="Str"(reference=w444, error in=w439, "Value"=w443) -> (error out=w441:errorcluster)  [unwired: 1 out]
          }
        }
      }
      frame "Handle Error" {
        n200 = Flush Queue(queue=w450, error in (no error)=w451) -> (queue out=w454:refnum<queue>, error out=w453:errorcluster)  [unwired: 1 out]
        n201 = Release Queue(queue=w454, force destroy? (F)=TRUE, error in (no error)=w453) -> (error out=w449:errorcluster)  [unwired: 2 out]
      }
    }
    "error out" <- w193
    "Numeric" <- w191
  }
  n202 = call "Destroy Client.vi"("error in"=w11, "gRPC ID"=w9) -> ("error out"=w10:errorcluster)  [unwired: 9 in]
  n203 = Unregister For Events(event registration refnum=w13, error in=w10) -> ()  [unwired: 1 out]
